vi "Read Single Analog Input.vi"(8 "error in (no error)":errorcluster, 10 "Parameter Name":string, 11 "Devices.DAQ Device":T2) -> (0 "error out":errorcluster, 2 "Analog Input Cluster":T1, 3 "data":dbl)   [LabVIEW 2021]
uses:
  <userlib>/DAQNavi Polymorphic VI/read/DAQNavi Read (Analog DBL 1Chan 1Samp).vi
  Analog Cluster.ctl
  <userlib>/DAQNavi Polymorphic VI/read/DAQNavi Read (Analog 2D DBL NChan NSamp).vi
  DAQNav Cluster.ctl
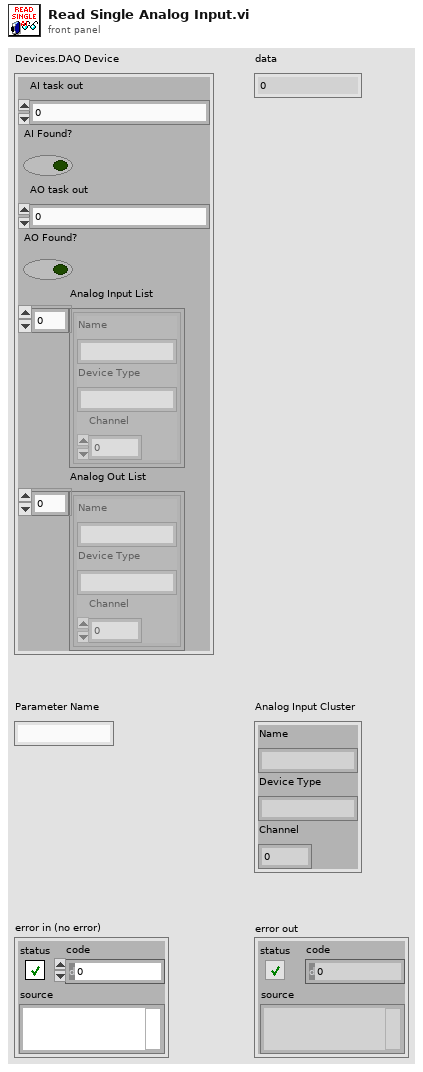
[diagram p1: front panel]
types:
  T1 = typedef "Analog Cluster.ctl" = cluster{"Name":string, "Device Type":string, "Channel":i32}
  T2 = typedef "DAQNav Cluster.ctl" = cluster{"AI task out":i32, "AI Found?":bool, "AO task out":i32, "AO Found?":bool, "Analog Input List":T1[], "Analog Out List":T1[]}
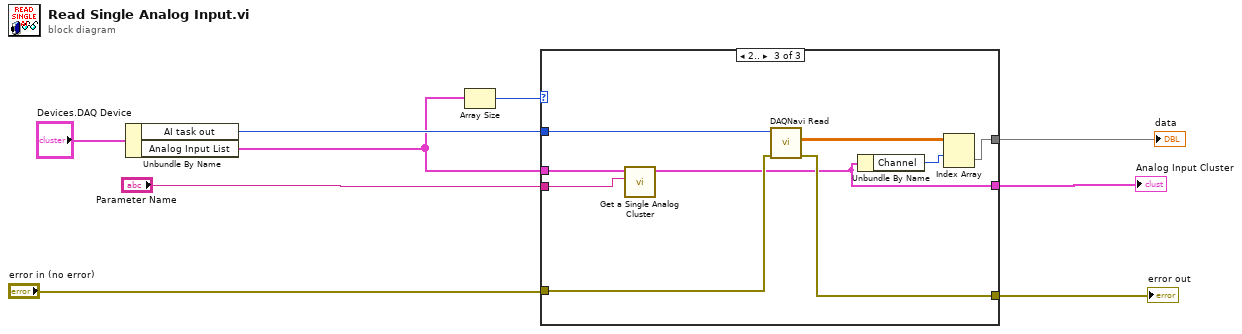
[diagram p0: block diagram]
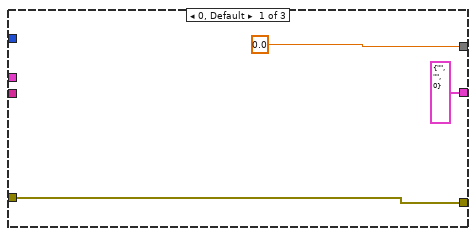
[diagram p2: hidden frame]
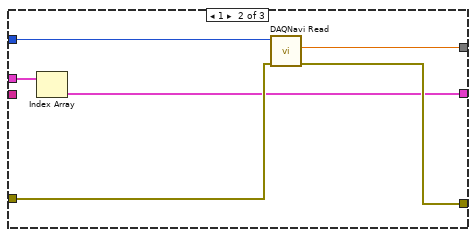
[diagram p3: hidden frame]
diagram:
  n1 = Unbundle By Name("Devices.DAQ Device") -> ("AI task out"=w7:i32, "Analog Input List"=w2:T1[])
  n2 = Array Size(array=w2) -> (size(s)=w6:i32)
  n3 = case shown="2.." w6 {
    tunnel: [0.0 ("data") w18 w22] -> w4
    tunnel: [w12 w17 w27] -> w9
    tunnel: w7 -> [_ w16 w26]
    tunnel: "error in (no error)" -> [w12 w15 w25]
    tunnel: "Parameter Name" -> [_ _ w21]
    tunnel: w2 -> [_ w14 w20]
    tunnel: [T1 {"Name"="", "Device Type"="", "Channel"=0} ("Analog Input Cluster") w13 w19] -> w1
    frame 0, Default {
    }
    frame 1 {
      n4 = Index Array(array=w14) -> (element=w13:T1)  [unwired: 1 in]
      n5 = call-poly <userlib>:"DAQNavi Read.vi"("error in (no error)"=w15, "task in"=w16) -> ("error out"=w17:errorcluster, "data"=w18:dbl)  [unwired: 7 in, 1 out]
    }
    frame 2.. {
      n6 = call "Get a Single Analog Cluster.vi"("Parameter Name"=w21, "Analog Input List"=w20) -> ("Analog Input Cluster"=w19:T1)  [unwired: 9 in]
      n7 = call-poly <userlib>:"DAQNavi Read.vi"("error in (no error)"=w25, "task in"=w26) -> ("error out"=w27:errorcluster, "data"=w24:dbl[][])  [unwired: 6 in, 2 out]
      n8 = Unbundle By Name(w19) -> ("Channel"=w23:i32)
      n9 = Index Array(array=w24, index (row)=w23) -> (element=w22:dbl[])  [unwired: 1 in]
    }
  }
  "data" <- w4
  "error out" <- w9
  "Analog Input Cluster" <- w1
